vi "RPLiDAR_C1.vi"() -> ()   [LabVIEW 2023]
uses:
  <vilib>/Analysis/coordinate.llb/2D Cartesian Coordinate Rotation (Array).vi
  5d9b0d3e-c3ec-43ca-bcc2-86a0b71de708.vi
  <vilib>/Instr/_visa.llb/VISA Configure Serial Port (Instr).vi
  <vilib>/Analysis/NI_AALPro.lvlib
panel:
  in  "탭 컨트롤":T1(tab)=enum."RAW DATA"
  in  "COM4 2":refnum<visa-resource-name>="COM12" caption="LiDAR_Com."
  out "read buffer":string
  out "ROI 그래프":cluster{dbl[], dbl[]}[](graph)=[{[-500.0, 500.0, 500.0, -500.0, -500.0], [0.0, 0.0, 1000.0, 1000.0, 0.0]}, {[], []}]
  in  "X MIN":dbl=-500.0
  in  "X MAX":dbl=500.0
  in  "Y MAX":dbl=1000.0
  in  "Y MIN":dbl
  out "DOWN":cluster{dbl[], dbl[]}[](graph)=[{[-500.0, 500.0, 500.0, -500.0, -500.0], [0.0, 0.0, 1000.0, 1000.0, 0.0]}, {[], []}]
  in  "GRID NUMBER":dbl=10.0
  out "CLUSTERED":T2(graph)=[{"array with duplicates removed"=[-500.0, 500.0, 500.0, -500.0, -500.0], "array with duplicates removed"=[0.0, 0.0, 1000.0, 1000.0, 0.0]}]
  in  "유클리디언":dbl=30.0
  in  "최대개수":i32=60
  in  "최소개수":i32=8
  out "Representative point":cluster{dbl[], dbl[]}[](graph)=[{[-500.0, 500.0, 500.0, -500.0, -500.0], [0.0, 0.0, 1000.0, 1000.0, 0.0]}, {[], []}]
  out "Loop Time":u32=93
  in  "Stop":bool
  # "RPLIDAR S2"
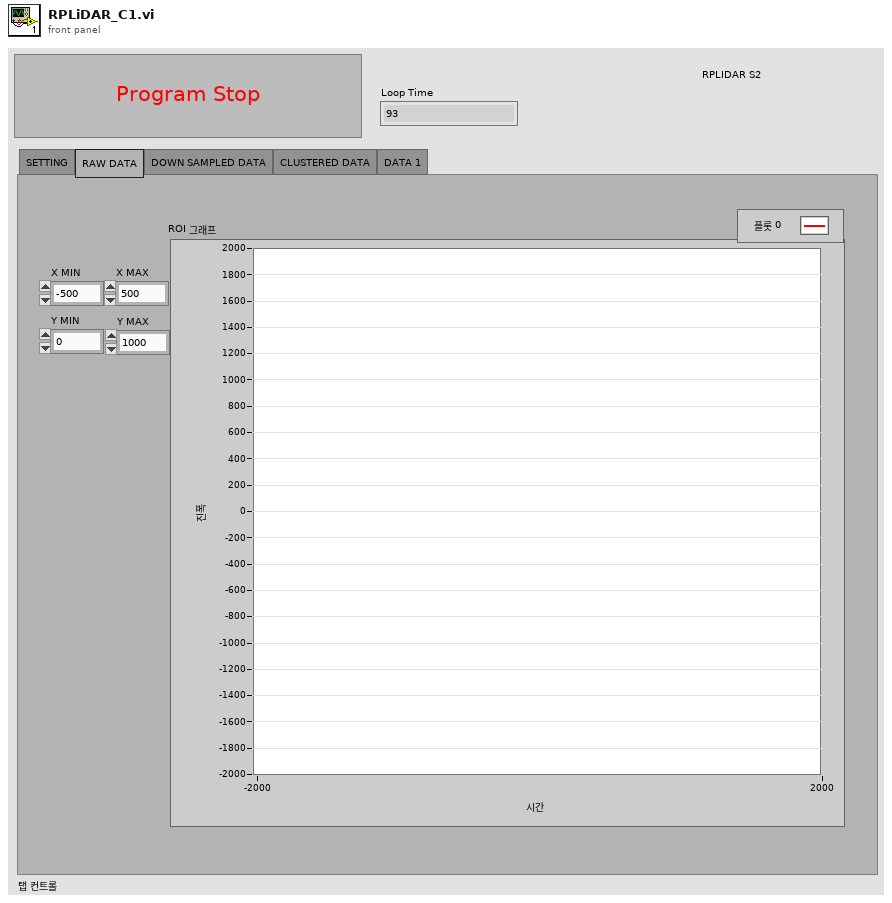
[diagram p1: front panel]
types:
  T1 = enum32{"SETTING", "RAW DATA", "DOWN SAMPLED DATA", "CLUSTERED DATA", "DATA 1"}
  T2 = cluster{"array with duplicates removed":dbl[], "array with duplicates removed":dbl[]}[]
  T3 = cluster{"array with duplicates removed":i32[], "array with duplicates removed":i32[]}
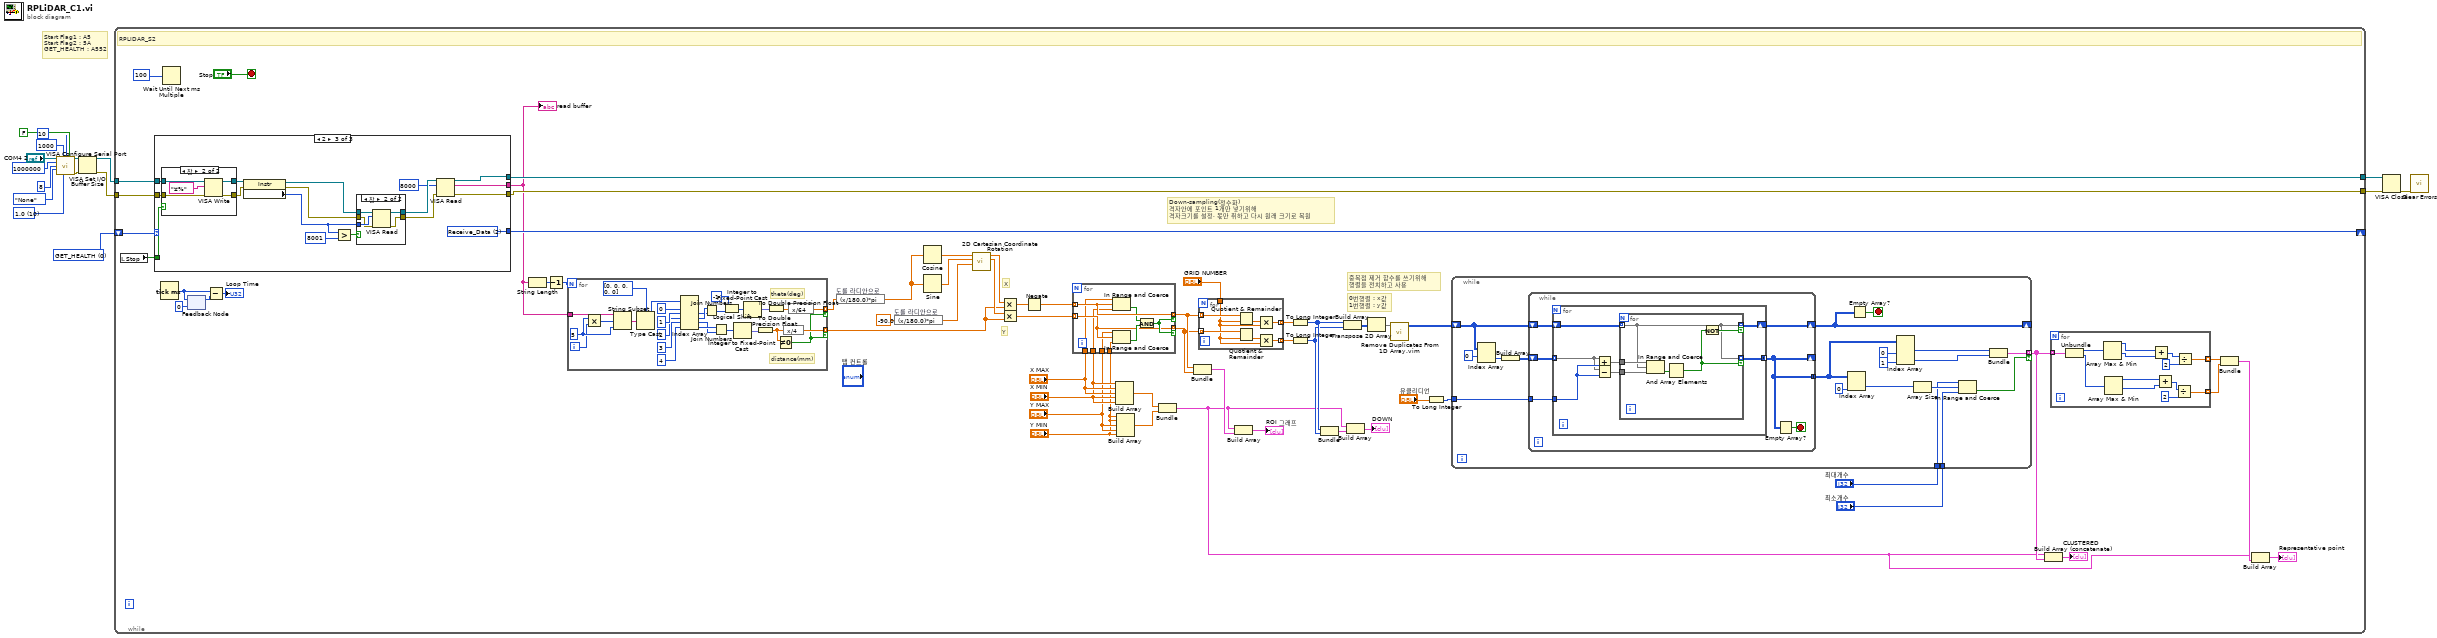
[diagram p0: block diagram]
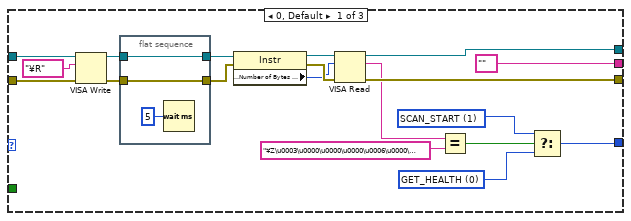
[diagram p2: hidden frame]
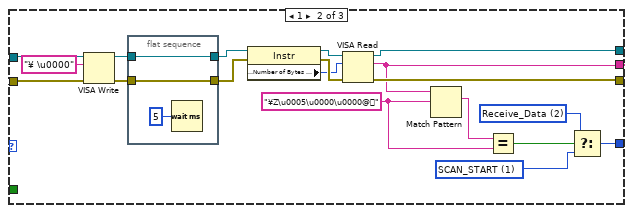
[diagram p3: hidden frame]
diagram:
  w1 = u16 10 items=["1.0"=10, "1.5"=15, "2.0"=20] ("stop bits (10: 1 bit)")
  w3 = u16 0 items=["GET_HEALTH", "SCAN_START", "Receive_Data"]
  # "Start Flag1 : A5\nStart Flag2 : 5A \nGET_HEALTH : A552"
  n1 = call-poly "VISA Configure Serial Port"("VISA resource name"="COM4 2", "timeout (10sec)"=u32 1000, "termination char\n(0xA = '\\n' = LF)"=u8 10 ("termination char\n(0xA = '\\n' = LF)"), "Enable Termination\nChar (T)"=FALSE ("Enable Termination\nChar (T)"), "baud rate (9600)"=u32 1000000, "data bits (8)"=u16 8, "parity (0:none)"=enum16{"None", "Odd", "Even", "Mark", "Space"}."None", "stop bits (10: 1 bit)"=w1) -> ("VISA resource name out"=w11:refnum<visa-resource-name>, "error out"=w10:errorcluster)  [unwired: 6 in]
  n2 = VISA Set I/O Buffer Size(VISA resource name=w11, error in (no error)=w10) -> (VISA resource name out=w5:refnum<visa-resource-name>, error out=w4:errorcluster)  [unwired: 2 in]
  n3 = while {
    tunnel: [w65] -> w15
    tunnel: [w66] -> w14
    tunnel: w5 -> [w74]
    tunnel: w4 -> [w73]
    shift-right: [w72] -> _
    shift-left: w3 -> [w75]
    stop <- "Stop" stop-if-true
    # "0번행렬 : x값\n1번행렬 : y값"
    # "중복점 제거 함수를 쓰기위해\n행렬을 전치하고 사용"
    # "Down-sampling(정수화)\n격자안에 포인트 1개만 넣기위해\n격자크기를 설정, 몫만 취하고 다시 원래 크기로 복원"
    # "Y"
    # "X"
    # "RPLIDAR_S2"
    n4 = local read "Stop"() -> (w71:bool)
    n5 = case shown="2" w75 {
      tunnel: w74 -> [w187 w205 w228]
      tunnel: w73 -> [w186 w204 w227]
      tunnel: [w188 w201 w214] -> w72
      tunnel: [w177 w202 w230] -> w66
      tunnel: [w176 w203 w229] -> w65
      tunnel: w71 -> [_ _ w226]
      tunnel: ["" ("read buffer") w199 w225] -> w47
      frame 0, Default {
        w170 = u16 0 items=["GET_HEALTH", "SCAN_START", "Receive_Data"]
        w171 = u16 1 items=["GET_HEALTH", "SCAN_START", "Receive_Data"]
        n6 = VISA Write(VISA resource name=w187, write buffer="¥R", error in (no error)=w186) -> (VISA resource name out=w181:refnum<visa-resource-name>, error out=w180:errorcluster)  [unwired: 1 out]
        n7 = flat-sequence {
          tunnel: w181 -> [w190]
          tunnel: w180 -> [w189]
          tunnel: [w190] -> w179
          tunnel: [w189] -> w178
          frame #0 {
            n8 = Wait (ms)(milliseconds to wait=u32 5 ("대기 시간 (ms)")) -> ()  [unwired: 1 out]
          }
        }
        n9 = property class="Instr"(reference=w179, error in=w178) -> (reference out=w184:refnum<visa-resource-name>, error out=w183:errorcluster, "Serial Settings:Number of Bytes at Serial Port"=w182:u32)
        n10 = VISA Read(VISA resource name=w184, byte count=w182, error in (no error)=w183) -> (VISA resource name out=w176:refnum<visa-resource-name>, read buffer=w173:string, error out=w177:errorcluster)  [unwired: 1 out]
        n11 = Equal?(x=w173, y="¥Z\u0003\u0000\u0000\u0000\u0006\u0000\u0000\u0000") -> (x = y?=w174:bool)
        n12 = Select(t=w171, s=w174, f=w170) -> (s? t:f=w188:u16)
      }
      frame 1 {
        w192 = u16 2 items=["GET_HEALTH", "SCAN_START", "Receive_Data"]
        w193 = u16 1 items=["GET_HEALTH", "SCAN_START", "Receive_Data"]
        w206 = "¥Z\u0005\u0000\u0000@"
        n13 = VISA Write(VISA resource name=w205, write buffer="¥ \u0000", error in (no error)=w204) -> (VISA resource name out=w208:refnum<visa-resource-name>, error out=w209:errorcluster)  [unwired: 1 out]
        n14 = flat-sequence {
          tunnel: w208 -> [w212]
          tunnel: w209 -> [w211]
          tunnel: [w212] -> w195
          tunnel: [w211] -> w194
          frame #0 {
            n15 = Wait (ms)(milliseconds to wait=u32 5 ("대기 시간 (ms)")) -> ()  [unwired: 1 out]
          }
        }
        n16 = property class="Instr"(reference=w195, error in=w194) -> (reference out=w198:refnum<visa-resource-name>, error out=w197:errorcluster, "Serial Settings:Number of Bytes at Serial Port"=w196:u32)
        n17 = VISA Read(VISA resource name=w198, byte count=w196, error in (no error)=w197) -> (VISA resource name out=w203:refnum<visa-resource-name>, read buffer=w199:string, error out=w202:errorcluster)  [unwired: 1 out]
        n18 = Match Pattern(string=w199, regular expression=w206) -> (match substring=w200:string)  [unwired: 1 in, 3 out]
        n19 = Equal?(x=w200, y=w206) -> (x = y?=w210:bool)
        n20 = Select(t=w192, s=w210, f=w193) -> (s? t:f=w201:u16)
      }
      frame 2 {
        w214 = u16 2 items=["GET_HEALTH", "SCAN_START", "Receive_Data"]
        n21 = case shown="참" w226 {
          tunnel: w228 -> [w239 w243]
          tunnel: w227 -> [w238 w242]
          tunnel: [w239 w241] -> w224
          tunnel: [w238 w240] -> w223
          frame False {
          }
          frame True {
            n22 = VISA Write(VISA resource name=w243, write buffer="¥%", error in (no error)=w242) -> (VISA resource name out=w241:refnum<visa-resource-name>, error out=w240:errorcluster)  [unwired: 1 out]
          }
        }
        n23 = property class="Instr"(reference=w224, error in=w223) -> (reference out=w219:refnum<visa-resource-name>, error out=w218:errorcluster, "Serial Settings:Number of Bytes at Serial Port"=w220:u32)
        n24 = Greater?(x=w220, y=u32 8001) -> (0:w222:bool)
        n25 = case shown="참" w222 {
          tunnel: w219 -> [w232 w237]
          tunnel: w220 -> [_ w236]
          tunnel: w218 -> [w231 w235]
          tunnel: [w232 w234] -> w217
          tunnel: [w231 w233] -> w216
          frame False {
          }
          frame True {
            n26 = VISA Read(VISA resource name=w237, byte count=w236, error in (no error)=w235) -> (VISA resource name out=w234:refnum<visa-resource-name>, error out=w233:errorcluster)  [unwired: 2 out]
          }
        }
        n27 = VISA Read(VISA resource name=w217, byte count=u32 8000, error in (no error)=w216) -> (VISA resource name out=w229:refnum<visa-resource-name>, read buffer=w225:string, error out=w230:errorcluster)  [unwired: 1 out]
      }
    }
    "read buffer" <- w47
    n28 = Tick Count (ms)() -> (millisecond timer value=w70:u32)
    n29 = Wait Until Next ms Multiple(millisecond multiple=u32 100 ("ms 배수")) -> ()  [unwired: 1 out]
    n30 = feedback #1(u32 0 ("millisecond timer value")) -> (w69:u32)
    n31 = feedback-in #1(w70) -> ()
    n32 = Subtract(x=w70, y=w69) -> (x-y=→"Loop Time":u32)
    n33 = String Length(string=w47) -> (length=w50:i32)
    n34 = Decrement(x=w50) -> (x-1=w51:i32)
    n35 = for {
      N: w51 -> [_]
      tunnel: [w143] -> w49 mode=indexing if=w146
      tunnel: [w147] -> w48 mode=indexing if=w146
      tunnel: w47 -> [w144]
      i -> [w149]
      w151 = 5 ("x")
      # "theta(deg)"
      # "distance(mm)"
      n36 = Multiply(x=w151, y=w149) -> (x*y=w136:i32)
      n37 = String Subset(string=w144, offset (0)=w136, length (rest)=w151) -> (substring=w152:string)
      n38 = Type Cast(type=u8[] [0, 0, 0, 0, 0], x=w152) -> (*(type *) &x=w150:u8[])
      n39 = Index Array(array=w150, index #1=0 ("index"), index #2=1 ("index"), index #3=2 ("index"), index #4=3 ("index"), index #5=4 ("index")) -> (element #2=w155:u8, element #3=w156:u8, element #4=w145:u8, element #5=w157:u8)  [unwired: 1 out]
      n40 = Join Numbers(hi=w156, lo=w155) -> ((hi.lo)=w154:u16)
      n41 = Join Numbers(hi=w157, lo=w145) -> ((hi.lo)=w153:u16)
      n42 = Logical Shift(y=i16 -1, x=w154) -> (x << y=w138:u16)
      n43 = Integer to Fixed-Point Cast(integer=w153) -> (fixed-point=w141:fxp<+,16,16>)  [unwired: 1 in]
      n44 = Integer to Fixed-Point Cast(integer=w138) -> (fixed-point=w142:fxp<+,16,16>)  [unwired: 1 in]
      n45 = To Double Precision Float(number=w141) -> (double precision float=w140:dbl)
      n46 = To Double Precision Float(number=w142) -> (double precision float=w139:dbl)
      n47 = Not Equal To 0?(x=w140) -> (x != 0?=w146:bool)
      n48 = expression code="x/4"(w140) -> (w147:dbl)
      n49 = expression code="x/64"(w139) -> (w143:dbl)
    }
    n50 = expression code="(x/180.0)*pi" "도를 라디안으로"(w49) -> (w58:dbl[])
    n51 = expression code="(x/180.0)*pi" "도를 라디안으로"(-90.0 ("theta")) -> (w52:dbl)
    n52 = Cosine(x=w58) -> (cos(x)=w57:dbl[])
    n53 = Sine(x=w58) -> (sin(x)=w56:dbl[])
    n54 = call-poly <vilib>:"2D Cartesian Coordinate Rotation.vi"("theta"=w52, "Y"=w56, "X"=w57) -> ("Y Out"=w53:dbl[], "X Out"=w54:dbl[])  [unwired: 6 in, 1 out]
    n55 = Multiply(x=w54, y=w48) -> (x*y=w46:dbl[])
    n56 = Multiply(x=w53, y=w48) -> (x*y=w32:dbl[])
    n57 = Negate(x=w46) -> (-x=w33:dbl[])
    n58 = for {
      tunnel: w33 -> [w97] mode=indexing
      tunnel: [w97] -> w31 mode=indexing if=w94
      tunnel: w32 -> [w93] mode=indexing
      tunnel: [w93] -> w30 mode=indexing if=w94
      tunnel: "X MAX" -> [w92]
      tunnel: "X MIN" -> [w91]
      tunnel: "Y MAX" -> [w90]
      tunnel: "Y MIN" -> [w89]
      n59 = In Range and Coerce(upper limit=w92, x=w97, lower limit=w91) -> (In Range?=w96:bool)  [unwired: 1 out]
      n60 = In Range and Coerce(upper limit=w90, x=w93, lower limit=w89) -> (In Range?=w95:bool)  [unwired: 1 out]
      n61 = And(x=w96, y=w95) -> (x .and. y?=w94:bool)
    }
    n62 = Build Array("X MIN", "X MAX", "X MAX", "X MIN", "X MIN") -> (w37:dbl[])
    n63 = Build Array("Y MIN", "Y MIN", "Y MAX", "Y MAX", "Y MIN") -> (w36:dbl[])
    n64 = Bundle(w37, w36) -> (w21:cluster{dbl[], dbl[]})  [unwired: 1 in]
    n65 = Bundle(w31, w30) -> (w35:cluster{dbl[], dbl[]})  [unwired: 1 in]
    n66 = for {
      tunnel: w31 -> [w169] mode=indexing
      tunnel: w30 -> [w168] mode=indexing
      tunnel: [w165] -> w63 mode=indexing
      tunnel: [w164] -> w64 mode=indexing
      tunnel: "GRID NUMBER" -> [w163]
      n67 = Quotient & Remainder(x=w169, y=w163) -> (floor(x/y)=w167:dbl)  [unwired: 1 out]
      n68 = Quotient & Remainder(x=w168, y=w163) -> (floor(x/y)=w166:dbl)  [unwired: 1 out]
      n69 = Multiply(x=w167, y=w163) -> (x*y=w165:dbl)
      n70 = Multiply(x=w166, y=w163) -> (x*y=w164:dbl)
    }
    n71 = Build Array(w21, w35) -> (→"ROI 그래프":cluster{dbl[], dbl[]}[])
    n72 = To Long Integer(number=w63) -> (32bit integer=w45:i32[])
    n73 = To Long Integer(number=w64) -> (32bit integer=w44:i32[])
    n74 = Bundle(w45, w44) -> (w28:cluster{i32[], i32[]})  [unwired: 1 in]
    n75 = Build Array(w45, w44) -> (w62:i32[][])
    n76 = Build Array(w21, w28) -> (→"DOWN":cluster{dbl[], dbl[]}[])
    n77 = Transpose 2D Array(2D array=w62) -> (transposed array=w60:i32[][])
    n78 = call "Remove Duplicates From 1D Array.vim"("array"=w60) -> ("array with duplicates removed"=w40:i32[][])  [unwired: 10 in]
    n79 = To Long Integer(number="유클리디언") -> (32bit integer=w42:i32)
    n80 = while {
      shift-right: [w110] -> _
      shift-left: w40 -> [w114]
      tunnel: w42 -> [w112]
      tunnel: [w111] -> w26 mode=indexing if=w100
      tunnel: "최소개수" -> [w107]
      tunnel: "최대개수" -> [w101]
      stop <- w109 stop-if-true
      n81 = Index Array(array=w114, index (row)=0 ("index")) -> (element=w115:i32[])  [unwired: 1 in]
      n82 = Build Array(w115) -> (w113:i32[][])
      n83 = while {
        shift-right: [w121] -> w110
        shift-left: w114 -> [w122]
        shift-right: [w117] -> _
        shift-left: w113 -> [w120]
        tunnel: w112 -> [w119]
        tunnel: [w117] -> w106 mode=concatenating
        stop <- w118 stop-if-true
        n84 = for {
          shift-right: [w128] -> w121
          shift-left: w122 -> [w129]
          tunnel: w120 -> [w123] mode=indexing
          tunnel: w119 -> [w124]
          tunnel: [w125] -> w117 mode=concatenating
          n85 = Add(x=w123, y=w124) -> (x+y=w127:i32[])
          n86 = Subtract(x=w123, y=w124) -> (x-y=w126:i32[])
          n87 = for {
            tunnel: w129 -> [w130] mode=indexing
            tunnel: [w130] -> w128 mode=indexing if=w133
            tunnel: w127 -> [w135]
            tunnel: w126 -> [w134]
            tunnel: [w130] -> w125 mode=indexing if=w131
            n88 = In Range and Coerce(upper limit=w135, x=w130, lower limit=w134) -> (In Range?=w132:bool[])  [unwired: 1 out]
            n89 = And Array Elements(Boolean array=w132) -> (logical AND=w131:bool)
            n90 = Not(x=w131) -> (.not. x?=w133:bool)
          }
        }
        n91 = Empty Array?(array=w117) -> (empty?=w118:bool)
      }
      n92 = Index Array(array=w106, index (col)=0 ("비활성화된 인덱스 (열)")) -> (element=w103:i32[])  [unwired: 1 in]
      n93 = Empty Array?(array=w110) -> (empty?=w109:bool)
      n94 = Index Array(array=w106, index (col) #1=0 ("인덱스 (행)"), index (col) #2=1 ("인덱스 (행)")) -> (element #1=w99:i32[], element #2=w98:i32[])  [unwired: 2 in]
      n95 = Array Size(array=w103) -> (size(s)=w102:i32)
      n96 = In Range and Coerce(upper limit=w101, x=w102, lower limit=w107) -> (In Range?=w100:bool)  [unwired: 1 out]
      n97 = Bundle("array with duplicates removed"=w99, "array with duplicates removed"=w98) -> (w111:T3)  [unwired: 1 in]
    }
    n98 = Build Array (concatenate)(w21, w26) -> (→"CLUSTERED":T2)
    n99 = for {
      tunnel: w26 -> [w88] mode=indexing
      tunnel: [w77] -> w25 mode=indexing
      tunnel: [w76] -> w24 mode=indexing
      n100 = Unbundle(w88) -> ("array with duplicates removed"=w87:i32[], "array with duplicates removed"=w86:i32[])
      n101 = Array Max & Min(array=w87) -> (max value=w85:i32, min value=w84:i32)  [unwired: 2 out]
      n102 = Array Max & Min(array=w86) -> (max value=w83:i32, min value=w82:i32)  [unwired: 2 out]
      n103 = Add(x=w85, y=w84) -> (x+y=w81:i32)
      n104 = Add(x=w83, y=w82) -> (x+y=w78:i32)
      n105 = Divide(x=w78, y=2) -> (x/y=w76:dbl)
      n106 = Divide(x=w81, y=2) -> (x/y=w77:dbl)
    }
    n107 = Bundle(w25, w24) -> (w23:cluster{dbl[], dbl[]})  [unwired: 1 in]
    n108 = Build Array(w21, w23) -> (→"Representative point":cluster{dbl[], dbl[]}[])
  }
  n109 = VISA Close(VISA resource name=w15, error in (no error)=w14) -> (error out=w16:errorcluster)
  n110 = call <vilib>:"Clear Errors.vi"("error in (no error)"=w16) -> ()  [unwired: 5 in, 2 out]
